vi "ReadBuffer4096.vi"(4 "string in":string, 5 "connection ID in":refnum<k5>) -> (0 "FIFO32_data":u32[](array[numeric]), 3 "connection ID out":refnum<k5>)   [LabVIEW 2020]
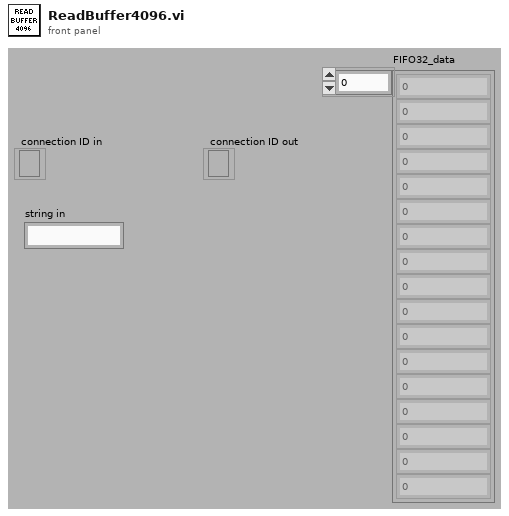
[diagram p1: front panel]
types:
  T1 = enum16{"Standard", "Buffered", "CRLF", "Immediate"}
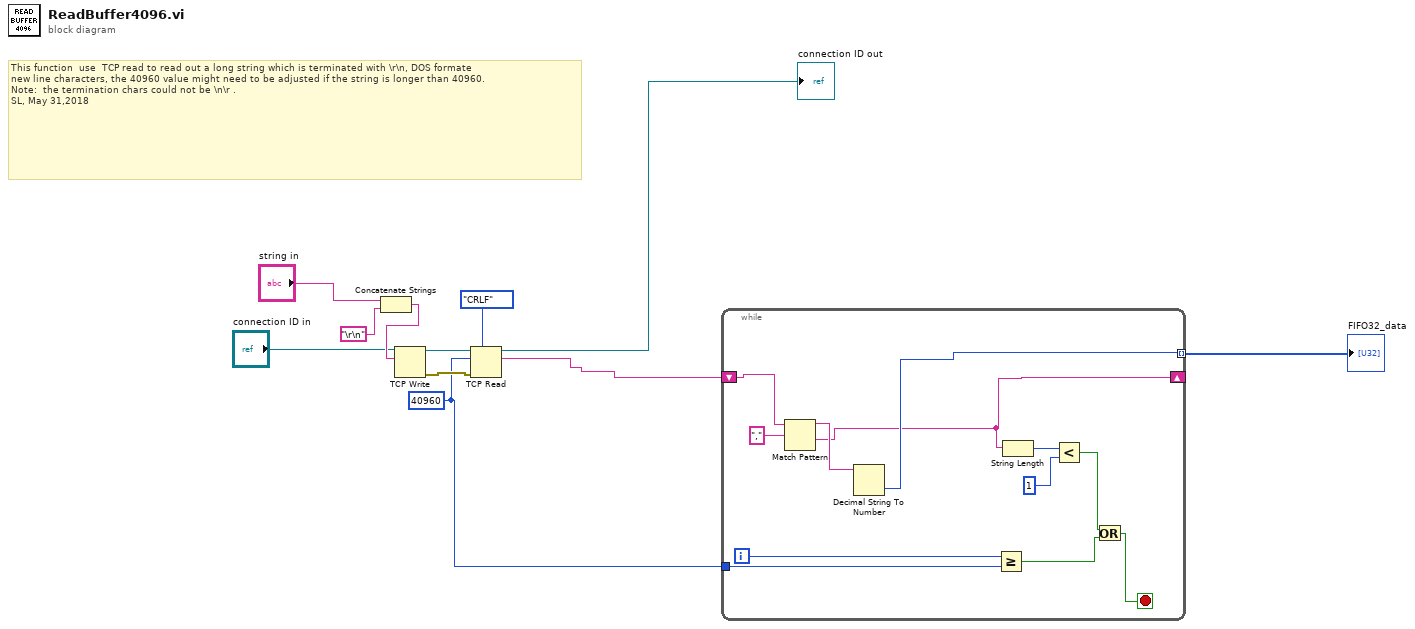
[diagram p0: block diagram]
diagram:
  w3 = 40960 ("bytes to read")
  # "This function  use  TCP read to read out a long string which is terminated with \\r\\n, DOS formate\nnew line characters, the 40960 value might need to be adjusted if the string is longer than 40960. \nNote:  the termination chars could not be \\n\\r . \nSL, May 31,2018"
  n1 = Concatenate Strings("string in", "\r\n") -> (w9:string)
  n2 = TCP Write(connection ID="connection ID in", data in=w9) -> (connection ID out=w11:refnum<k5>, error out=w4:errorcluster)  [unwired: 2 in, 1 out]
  n3 = TCP Read(connection ID=w11, bytes to read=w3, error in (no error)=w4, 7:T1."CRLF" ("mode (standard)")) -> (connection ID out=→"connection ID out":refnum<k5>, data out=w2:string)  [unwired: 1 in, 1 out]
  n4 = while {
    shift-right: [w15] -> _
    shift-left: w2 -> [w22]
    tunnel: [w21] -> w1 mode=indexing
    tunnel: w3 -> [w18]
    i -> [w19]
    stop <- w16 stop-if-true
    n5 = Match Pattern(string=w22, regular expression=",") -> (before substring=w20:string, after substring=w15:string)  [unwired: 1 in, 2 out]
    n6 = Decimal String To Number(string=w20) -> (number=w21:i32)  [unwired: 2 in, 1 out]
    n7 = Greater Or Equal?(x=w19, y=w18) -> (x >= y?=w17:bool)
    n8 = String Length(string=w15) -> (length=w14:i32)
    n9 = Less?(x=w14, y=1 ("bytes to read")) -> (x < y?=w12:bool)
    n10 = Or(x=w12, y=w17) -> (x .or. y?=w16:bool)
  }
  "FIFO32_data" <- w1
